vi "work1_GetOrder.vi"() -> ()   [LabVIEW 2026]
panel:
  out "Client counter":i32
  out "Order ID":i32
  in  "ID":i32
  in  "stop":bool
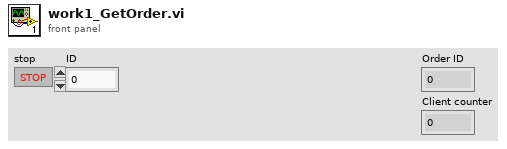
[diagram p1: front panel]
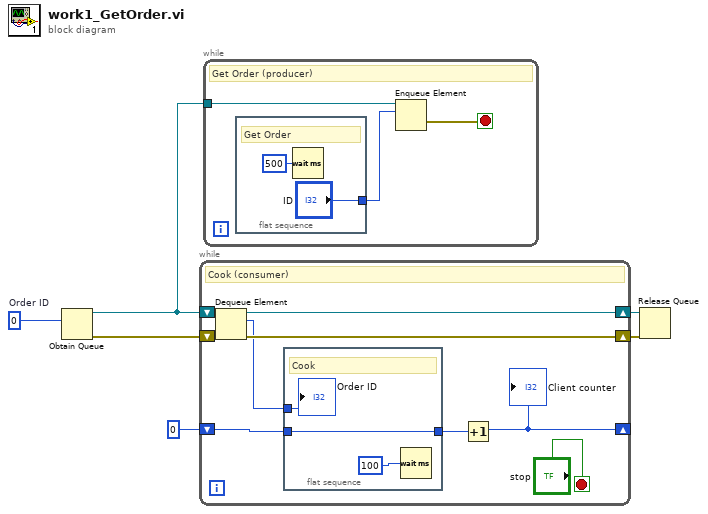
[diagram p0: block diagram]
diagram:
  w2 = 0  # Order ID
  n1 = Obtain Queue(element data type=w2) -> (queue out=w3:refnum<queue>, error out=w5:errorcluster)  [unwired: 4 in, 1 out]
  n2 = while {
    shift-right: [w13] -> w4
    shift-left: w5 -> [w14]
    shift-right: [w15] -> w6
    shift-left: w3 -> [w12]
    shift-right: [w9] -> _
    shift-left: u16 0 -> [w7]
    stop <- "stop" stop-if-true
    # "Cook (consumer)"
    n3 = Dequeue Element(queue=w12, error in (no error)=w14) -> (queue out=w15:refnum<queue>, element=w10:i32, error out=w13:errorcluster)  [unwired: 1 in, 1 out]
    n4 = flat-sequence {
      tunnel: w10 -> [w17]
      tunnel: [w16] -> w8
      tunnel: w7 -> [w16]
      frame #0 {
        # "Cook"
        n5 = Wait (ms)(milliseconds to wait=u32 100) -> ()  [unwired: 1 out]
        "Order ID" <- w17
      }
    }
    n6 = Increment(x=w8) -> (x+1=w9:u16)
    "Client counter" <- w9
  }
  n7 = while {
    tunnel: w3 -> [w21]
    stop <- w20 stop-if-true
    # "Get Order (producer)"
    n8 = flat-sequence {
      tunnel: ["ID"] -> w19
      frame #0 {
        # "Get Order"
        n9 = Wait (ms)(milliseconds to wait=u32 500) -> ()  [unwired: 1 out]
      }
    }
    n10 = Enqueue Element(queue=w21, element=w19) -> (error out=w20:errorcluster)  [unwired: 2 in, 2 out]
  }
  n11 = Release Queue(queue=w6, error in (no error)=w4) -> ()  [unwired: 1 in, 3 out]
